vi "Read name.vi"(8 "error in":errorcluster, 11 "PL_Local Target Configuration in":refnum<class "PL_Target Configuration.lvclass">) -> (0 "error out":errorcluster, 2 "name":string, 3 "PL_Local Target Configuration out":refnum<class "PL_Target Configuration.lvclass">)   [LabVIEW 2013, in "PL_Target Configuration.lvclass"]
uses:
  PL_Target Configuration.lvclass
  <vilib>/NI/Configuration Framework/serializable configuration/NISE_CEF_serializable configuration.lvclass
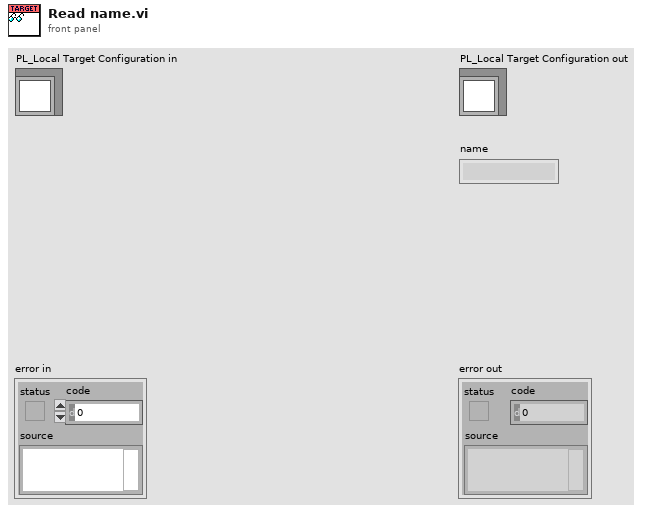
[diagram p1: front panel]
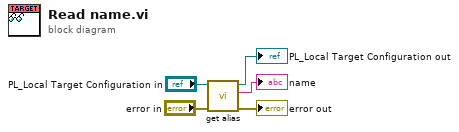
[diagram p0: block diagram]
diagram:
  n1 = call <vilib>:"get alias.vi"("error in"="error in", "configuration in"="PL_Local Target Configuration in") -> ("error out"=→"error out":errorcluster, "alias"=→"name":string, "configuration out"=→"PL_Local Target Configuration out":refnum<class "PL_Target Configuration.lvclass">)  [unwired: 7 in]
